vi "Close Project.vi"(8 "error in (no error)":errorcluster, 10 "Project Path in":path) -> (0 "error out":errorcluster, 2 "Project Path out":path)   [LabVIEW 2019, in "gRPC Template Creation Utility.lvlib"]
uses:
  gRPC Template Creation Utility.lvlib
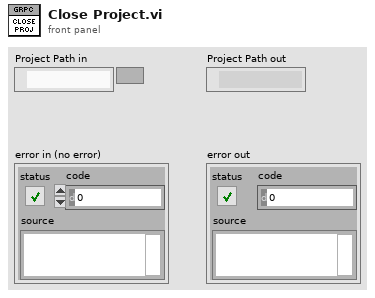
[diagram p1: front panel]
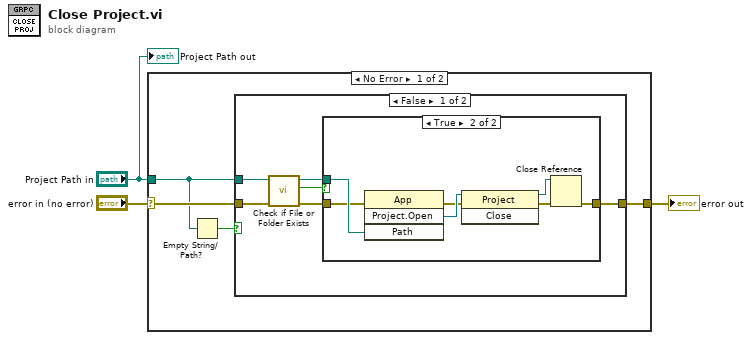
[diagram p0: block diagram]
diagram:
  n1 = case shown="No Error" "error in (no error)" {
    selector: "error in (no error)" -> [w6 w23]
    tunnel: "Project Path in" -> [w5 _]
    tunnel: [w7 w23] -> w2
    frame No Error {
      n2 = Empty String/Path?(string/path=w5) -> (empty?=w4:bool)
      n3 = case shown="False" w4 {
        tunnel: w5 -> [w13 _]
        tunnel: [w10 w22] -> w7
        tunnel: w6 -> [w9 w22]
        frame False {
          n4 = call <vilib>:"Check if File or Folder Exists.vi"("error in (no error)"=w9, "path"=w13) -> ("error out"=w11:errorcluster, "file or folder exists?"=w8:bool, "dup path"=w12:path)  [unwired: 7 in]
          n5 = case shown="True" w8 {
            tunnel: w12 -> [_ w21]
            tunnel: w11 -> [w14 w20]
            tunnel: [w14 w15] -> w10
            frame False {
            }
            frame True {
              n6 = invoke class="App" method="Project.Open"(error in=w20, "Path"=w21) -> (error out=w18:errorcluster, "Project:Open"=w19:refnum<vi>)  [unwired: 2 in, 2 out]
              n7 = invoke class="Project" method="Close"(reference=w19, error in=w18) -> (reference out=w16:refnum<vi>, error out=w17:errorcluster)  [unwired: 1 in, 1 out]
              n8 = Close Reference(reference=w16, error in (no error)=w17) -> (error out=w15:errorcluster)
            }
          }
        }
        frame True {
        }
      }
    }
    frame Error {
    }
  }
  "error out" <- w2
  "Project Path out" <- "Project Path in"
